vi "ImplementInterface.vi"(5 "AddInterfaceToClass(If not you still might want to create methods)":bool=TRUE, 6 "InterfaceMethodsToCreate":string[](array[string])=["Add.Vi", "Execute.vi"], 7 "ClassWriter.lvclass":refnum<class "ClassWriter.lvclass">, 8 "error in":errorcluster, 9 "CreateMethods":bool=TRUE, 10 "Interface Path":path=path "C:/Projects/Interface/Sub_Interface1/Sub_Interface1.lvclass", 11 "LvClassPath/LvClassProjectItem":variant) -> (0 "error out":errorcluster={"status"=TRUE, "code"=7, "source"="Invoke Node in InterfaceLibrary.lvlib:ImplementInterface.vi\n<APPEND>\nMethod Name: <b>LabVIEW Class:Open</b>"})   [LabVIEW 2020, in "InterfaceLibrary.lvlib"]
uses:
  InterfaceLibrary.lvlib
  Provider_BaseClassInterface/ClassWriter_class/ClassWriter.lvclass
  Provider_LvNativeClass/ClassWriterNative_class/ClassWriterNative.lvclass
  API/GDSAPI_SubVIs/GDSAPI_MethodType.ctl
  Provider_BaseClassInterface/CreateMethodData.ctl
  Provider_EndevoGOOP300/GOOP300_SubVIs/GOOP300_MethodScopeType.ctl
  Provider_LvNativeClass/ClassWriterNative_class/IconDetails.ctl
  Provider_LvNativeClass/ClassWriterNative_class/IconSize.ctl
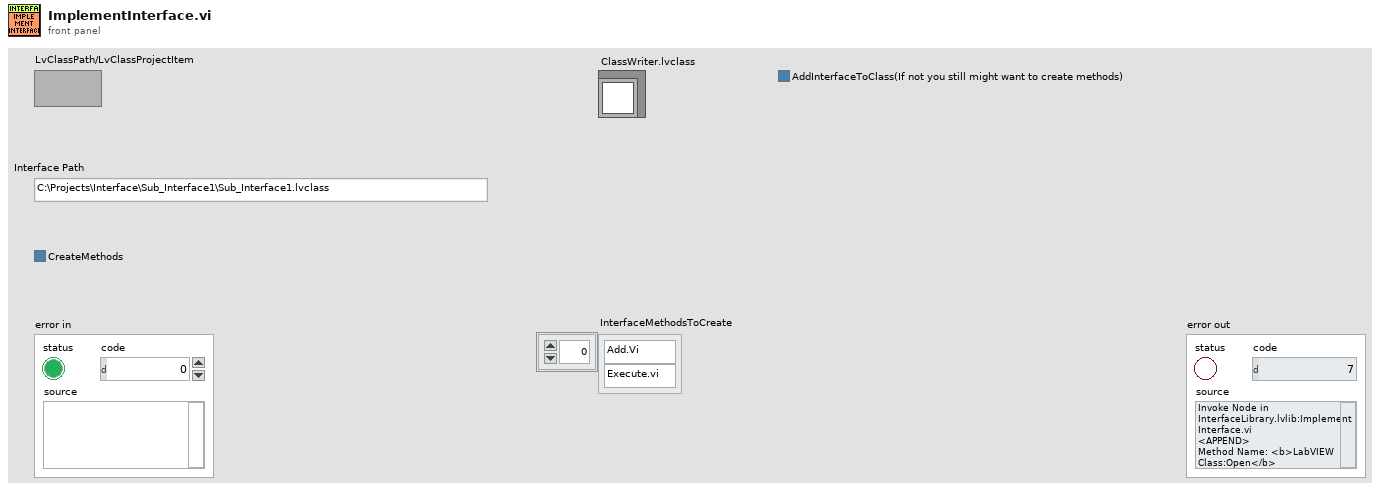
[diagram p1: front panel]
types:
  T1 = cluster{"ClassRef":refnum<vi>, "ClassRefCreated":bool, "Application":refnum<vi>, "InterfaceRef":refnum<vi>, "MethodsToImplement":path[], "MethodsDescription":string[], "MethodsScope":enum32{"invalid scope", "public", "private", "protected", "community"}[]}
  T2 = enum32{"invalid scope", "public", "private", "protected", "community"}
  T3 = typedef "GDSAPI_MethodType.ctl" = enum16{"Read Attribute", "Write Attribute", "Read & Write Attribute", "None Modifying Method", "Get Property", "Set Property", "Read Property", "Write Property", "Static Method", "Interface Method"}
  T4 = typedef "ClassWriter.lvclass/CreateMethodData.ctl" = cluster{"MethodName":string, "RelativeMethodPath":path, "MethodDescription":string, "Scope/Visibility":T5, "MethodTemplateName":string, "IconOut":u8[][], "RelativeProjectClassPath":string, "OpenViAfterCreation":bool, "DynamicDispatchVi":bool, "ExtraCreateParameters":variant, "MustOverride":bool, "MustCallParent":bool, "IconDetails":T6, "AF-Option":variant, "TemplatePath":path}
  T5 = typedef "GOOP300_MethodScopeType.ctl" = enum16{"Use Parent Folder Scope", "Public", "Protected", "Private", "Community"}
  T6 = typedef "ClassWriterNative.lvclass/IconDetails.ctl" = cluster{"IconSize":T7, "ImageRows(32)":i32, "ConnectorPaneHeight":i32[]}
  T7 = typedef "ClassWriterNative.lvclass/IconSize.ctl" = enum16{"Full", "1 c-term high", "2 c-term high", "3 c-term high"}
  T8 = enum32{"invalid scope", "public", "private", "protected", "community"}[]
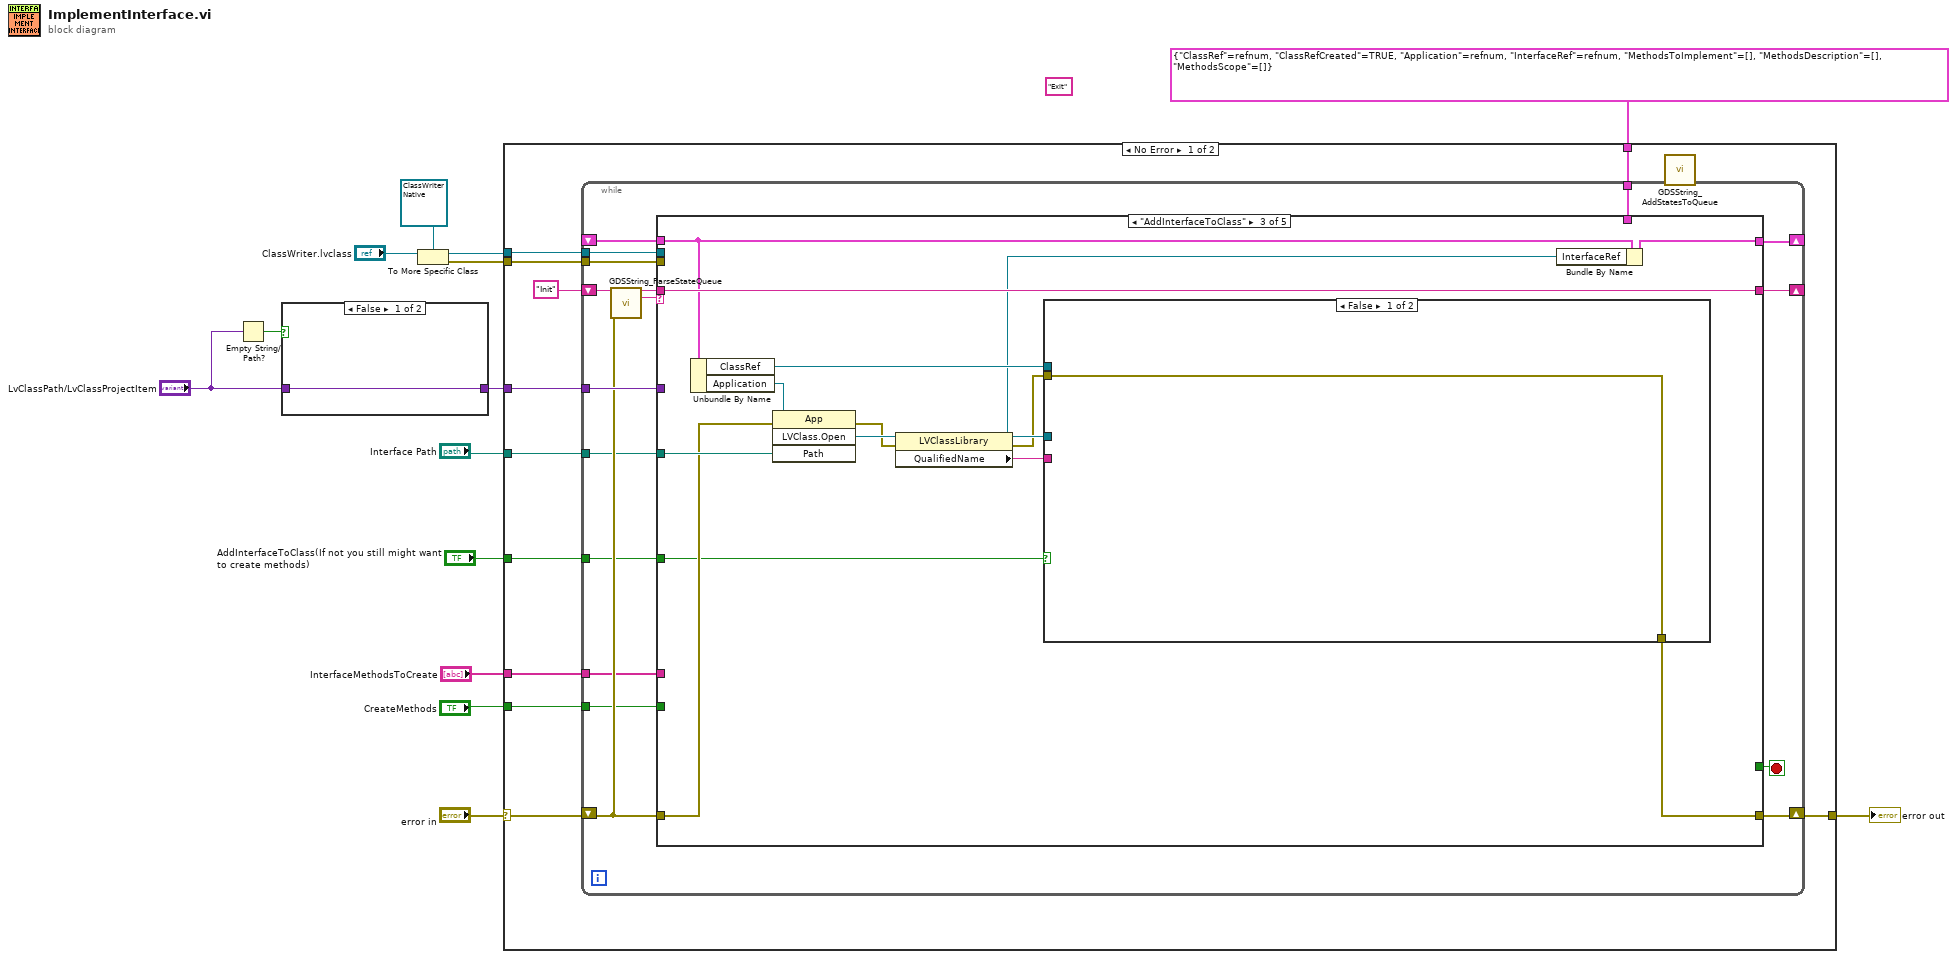
[diagram p0: block diagram]
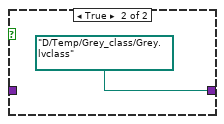
[diagram p2: hidden frame]
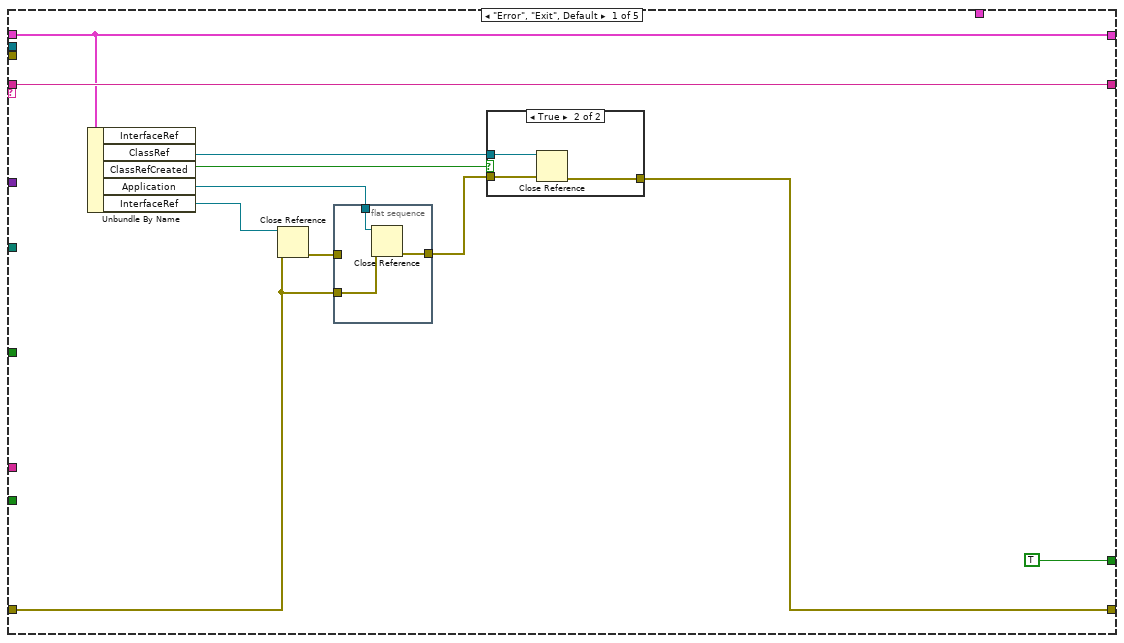
[diagram p3: hidden frame]
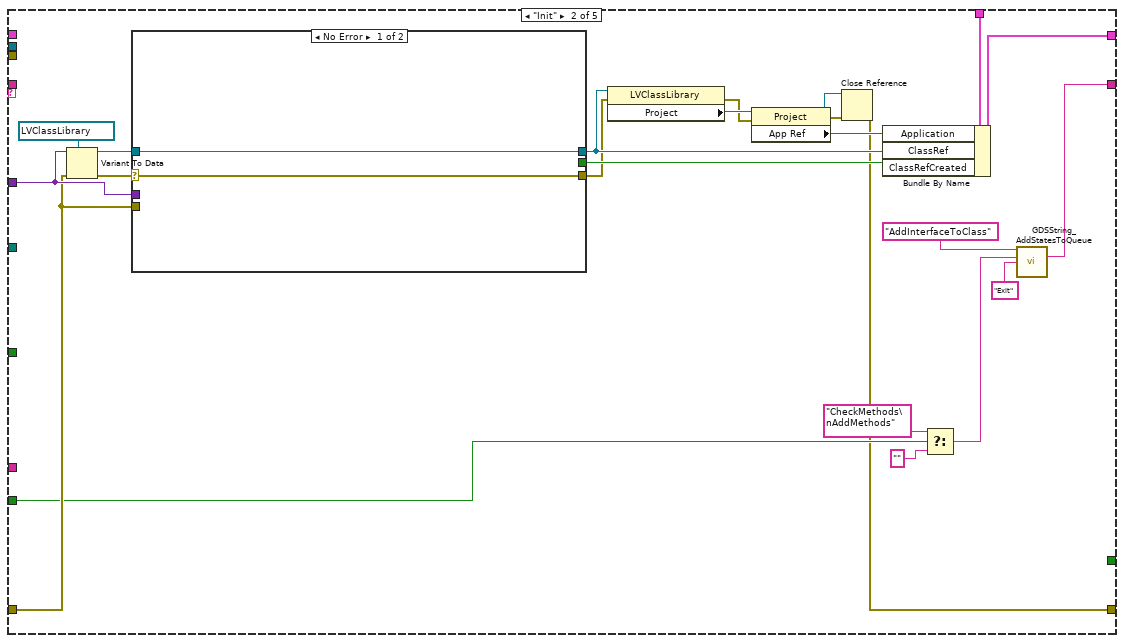
[diagram p5: hidden frame]
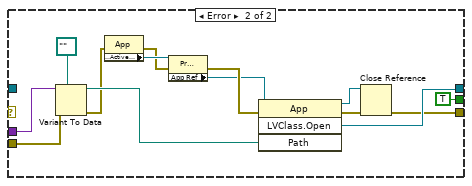
[diagram p6: hidden frame]
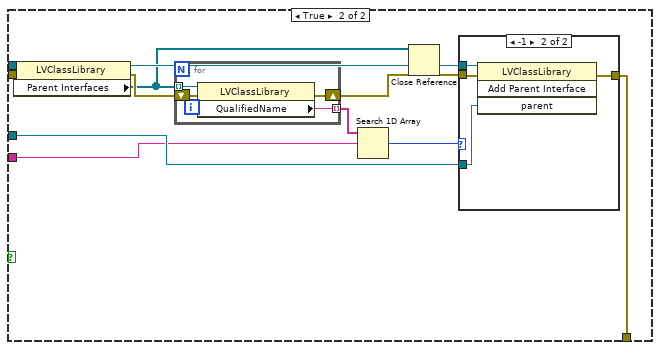
[diagram p7: hidden frame]
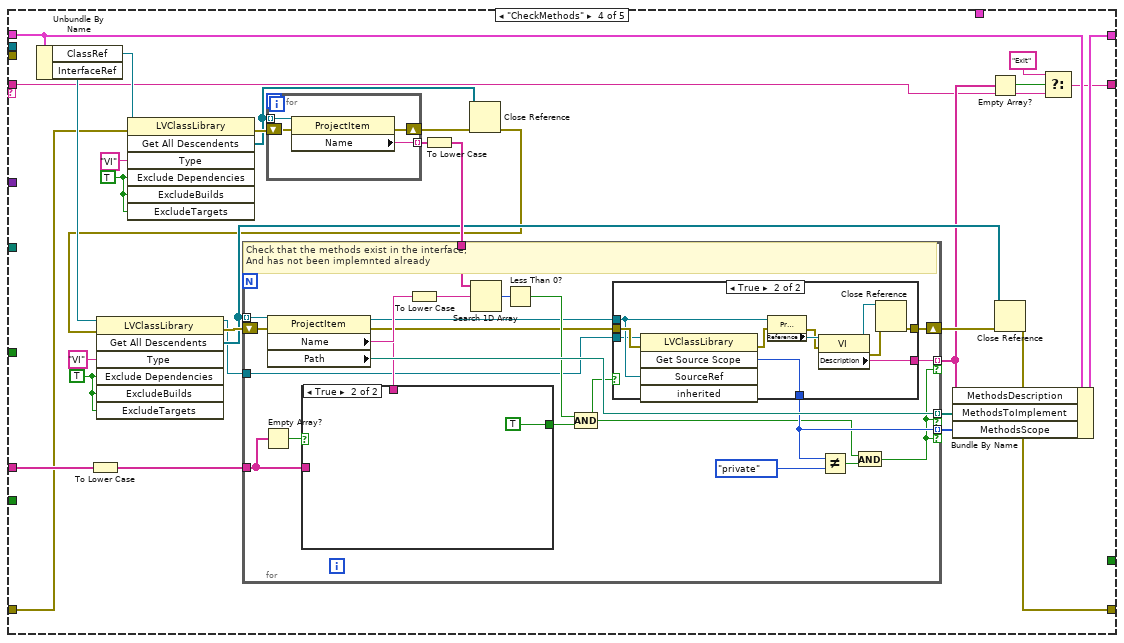
[diagram p9: hidden frame]
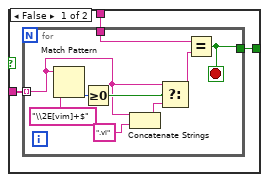
[diagram p11: hidden frame]
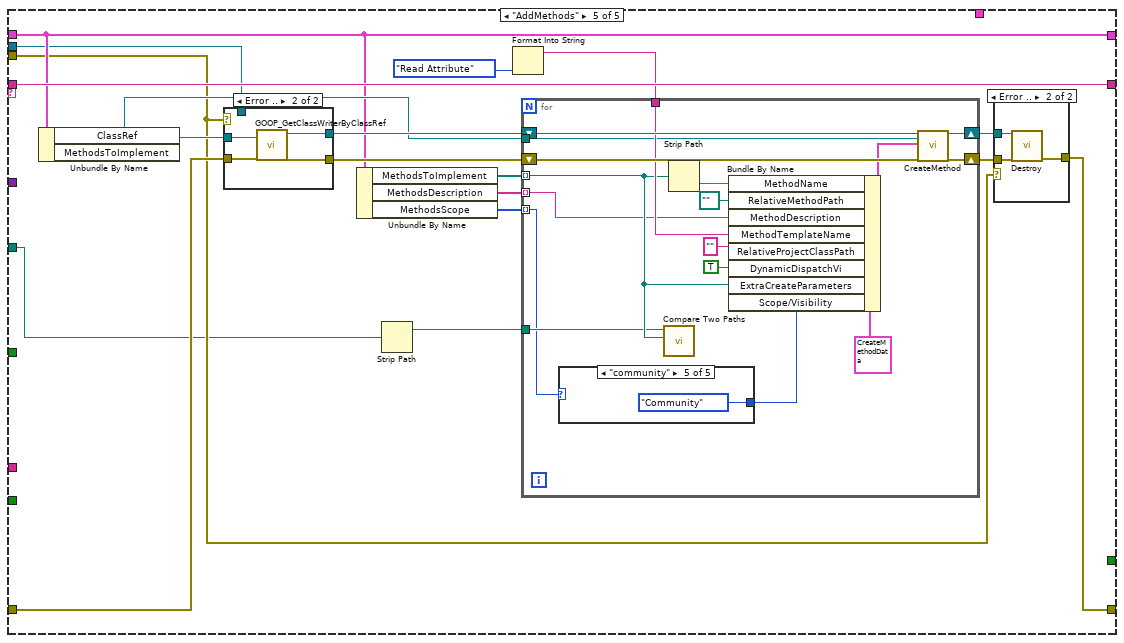
[diagram p12: hidden frame]
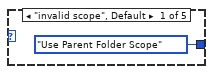
[diagram p15: hidden frame]
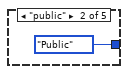
[diagram p16: hidden frame]
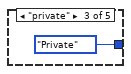
[diagram p17: hidden frame]
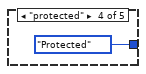
[diagram p18: hidden frame]
diagram:
  (unwired) "Exit" ("Remaining States")
  n1 = Empty String/Path?(string/path="LvClassPath/LvClassProjectItem") -> (empty?=w10:bool)
  n2 = case shown="False" w10 {
    tunnel: "LvClassPath/LvClassProjectItem" -> [w15 _]
    tunnel: [w15 path "D:/Temp/Grey_class/Grey.lvclass" ("Path")] -> w8
    frame False {
    }
    frame True {
    }
  }
  n3 = To More Specific Class(target class=refnum<class "ClassWriterNative.lvclass"> refnum ("ClassWriterNative"), reference="ClassWriter.lvclass") -> (specific class reference=w4:refnum<class "ClassWriterNative.lvclass">, error out=w2:errorcluster)  [unwired: 1 in]
  n4 = case shown="No Error" "error in" {
    selector: "error in" -> [w26 w267]
    tunnel: w8 -> [w27 _]
    tunnel: [w25 w267] -> w13
    tunnel: T1 {"ClassRef"=refnum, "ClassRefCreated"=TRUE, "Application"=refnum, "InterfaceRef"=refnum, "MethodsToImplement"=[], "MethodsDescription"=[], "MethodsScope"=[]} -> [w23 _]
    tunnel: "CreateMethods" -> [w22 _]
    tunnel: "Interface Path" -> [w21 _]
    tunnel: "InterfaceMethodsToCreate" -> [w20 _]
    tunnel: w4 -> [w19 _]
    tunnel: w2 -> [w18 _]
    tunnel: "AddInterfaceToClass(If not you still might want to create methods)" -> [w17 _]
    frame No Error {
      n5 = while {
        tunnel: w27 -> [w44]
        shift-right: [w43] -> w25
        shift-left: w26 -> [w41]
        shift-right: [w35] -> _
        shift-left: "Init" -> [w42]
        tunnel: w23 -> [w39]
        shift-right: [w38] -> _
        shift-left: _ -> [w37]
        tunnel: w22 -> [w33]
        tunnel: w21 -> [w32]
        tunnel: w20 -> [w31]
        tunnel: w19 -> [w30]
        tunnel: w18 -> [w29]
        tunnel: w17 -> [w28]
        stop <- w34 stop-if-true
        n6 = call "GDSString_ParseStateQueue.vi"("State Queue"=w42, "Error In (no error)"=w41) -> ("Remaining States"=w36:string, "Current State"=w40:string)  [unwired: 9 in, 3 out]
        n7 = case shown="\"AddInterfaceToClass\"" w40 {
          tunnel: w44 -> [_ w82 _ _ _]
          tunnel: w41 -> [w45 w81 w109 w145 w225]
          tunnel: [w48 w65 w110 w146 w229] -> w43
          tunnel: [w53 w79 w108 w155 w223] -> w38
          tunnel: w39 -> [_ w80 _ _ _]
          tunnel: w37 -> [w53 _ w114 w164 w223]
          tunnel: [w55 w77 w115 w153 w234] -> w35
          tunnel: w36 -> [w55 _ w115 w142 w234]
          tunnel: [TRUE _ _ _ _] -> w34
          tunnel: w33 -> [_ w76 _ _ _]
          tunnel: w32 -> [_ _ w111 _ w217]
          tunnel: w31 -> [_ _ _ w159 _]
          tunnel: w30 -> [_ _ _ _ w219]
          tunnel: w29 -> [_ _ _ _ w220]
          tunnel: w28 -> [_ _ w102 _ _]
          frame "Error", "Exit", Default {
            n8 = Unbundle By Name(w53) -> ("ClassRef"=w51:refnum<vi>, "ClassRefCreated"=w52:bool, "Application"=w50:refnum<vi>, "InterfaceRef"=w47:refnum<vi>)  [unwired: 1 out]
            n9 = Close Reference(reference=w47, error in (no error)=w45) -> (error out=w46:errorcluster)
            n10 = flat-sequence {
              tunnel: w50 -> [w58]
              tunnel: [w57] -> w49
              tunnel: w46 -> [_]
              tunnel: w45 -> [w56]
              frame #0 {
                n11 = Close Reference(reference=w58, error in (no error)=w56) -> (error out=w57:errorcluster)
              }
            }
            n12 = case shown="True" w52 {
              tunnel: w51 -> [_ w62]
              tunnel: w49 -> [w59 w61]
              tunnel: [w59 w60] -> w48
              frame False {
              }
              frame True {
                n13 = Close Reference(reference=w62, error in (no error)=w61) -> (error out=w60:errorcluster)
              }
            }
          }
          frame "Init" {
            n14 = Variant To Data(error in=w81, type=refnum<vi> refnum ("ProjectItem"), Variant=w82) -> (data=w84:refnum<vi>, error out=w83:errorcluster)
            n15 = case shown="No Error" w83 {
              selector: w83 -> [w86 _]
              tunnel: w84 -> [w87 _]
              tunnel: [w86 w93] -> w66
              tunnel: w82 -> [_ w100]
              tunnel: w81 -> [_ w97]
              tunnel: [w87 w96] -> w70
              tunnel: [_ TRUE] -> w78
              frame No Error {
              }
              frame Error {
                n16 = Variant To Data(error in=w97, type=path "" ("Path"), Variant=w100) -> (data=w99:path, error out=w98:errorcluster)
                n17 = property class="App"(error in=w98) -> (error out=w90:errorcluster, "Project.ActiveProject"=w91:refnum<vi>)  [unwired: 1 in, 1 out]
                n18 = property class="Project"(reference=w91, error in=w90) -> (error out=w89:errorcluster, "App Ref"=w88:refnum<vi>)  [unwired: 1 out]
                n19 = invoke class="App" method="LVClass.Open"(reference=w88, error in=w89, "Path"=w99) -> (reference out=w94:refnum<vi>, error out=w95:errorcluster, "LVClass.Open"=w96:refnum<vi>)  [unwired: 1 in, 1 out]
                n20 = Close Reference(reference=w94, error in (no error)=w95) -> (error out=w93:errorcluster)
              }
            }
            n21 = property class="LVClassLibrary"(reference=w70, error in=w66) -> (error out=w63:errorcluster, "Project"=w64:refnum<vi>)  [unwired: 1 out]
            n22 = property class="Project"(reference=w64, error in=w63) -> (reference out=w68:refnum<vi>, error out=w67:errorcluster, "App Ref"=w69:refnum<vi>)
            n23 = Close Reference(reference=w68, error in (no error)=w67) -> (error out=w65:errorcluster)
            n24 = Bundle By Name(cluster=w80, "Application"=w69, "ClassRef"=w70, "ClassRefCreated"=w78) -> (w79:T1)
            n25 = Select(t="CheckMethods\nAddMethods" ("Remaining States"), s=w76, f="") -> (s? t:f=w72:string)
            n26 = call "GDSString_AddStatesToQueue.vi"("State(s) in Front (\"\")"="AddInterfaceToClass" ("Remaining States"), "State(s) in (\"\")"=w72, "State(s) at Back (\"\")"="Exit" ("Remaining States")) -> ("States Out"=w77:string)  [unwired: 12 in]
          }
          frame "AddInterfaceToClass" {
            n27 = Unbundle By Name(w114) -> ("ClassRef"=w113:refnum<vi>, "Application"=w112:refnum<vi>)
            n28 = invoke class="App" method="LVClass.Open"(reference=w112, error in=w109, "Path"=w111) -> (error out=w104:errorcluster, "LVClass.Open"=w107:refnum<vi>)  [unwired: 1 in, 2 out]
            n29 = property class="LVClassLibrary"(reference=w107, error in=w104) -> (reference out=w106:refnum<vi>, error out=w103:errorcluster, "QualifiedName"=w105:string)
            n30 = case shown="False" w102 {
              tunnel: w113 -> [_ w128]
              tunnel: [w116 w125] -> w110
              tunnel: w106 -> [_ w124]
              tunnel: w105 -> [_ w123]
              tunnel: w103 -> [w116 w122]
              frame False {
              }
              frame True {
                n31 = property class="LVClassLibrary"(reference=w128, error in=w122) -> (reference out=w126:refnum<vi>, error out=w121:errorcluster, "Parent Interfaces"=w117:refnum<vi>[])
                n32 = for {
                  tunnel: w117 -> [w132] mode=indexing
                  tunnel: [w131] -> w120 mode=indexing
                  shift-right: [w130] -> w119
                  shift-left: w121 -> [w129]
                  n33 = property class="LVClassLibrary"(reference=w132, error in=w129) -> (error out=w130:errorcluster, "QualifiedName"=w131:string)  [unwired: 1 out]
                }
                n34 = Search 1D Array(1D array=w120, element=w123) -> (index of element=w127:i32)  [unwired: 1 in]
                n35 = Close Reference(reference=w117, error in (no error)=w119) -> (error out=w118:errorcluster)
                n36 = case shown="-1" w127 {
                  tunnel: w126 -> [_ w137]
                  tunnel: w118 -> [w133 w136]
                  tunnel: w124 -> [_ w135]
                  tunnel: [w133 w134] -> w125
                  frame 0, Default {
                  }
                  frame -1 {
                    n37 = invoke class="LVClassLibrary" method="Add Parent Interface"(reference=w137, error in=w136, "parent"=w135) -> (error out=w134:errorcluster)  [unwired: 1 in, 3 out]
                  }
                }
              }
            }
            n38 = Bundle By Name(cluster=w114, "InterfaceRef"=w106) -> (w108:T1)
          }
          frame "CheckMethods" {
            w162 = TRUE ("ExcludeDependencies")
            w165 = TRUE ("ExcludeDependencies")
            n39 = Unbundle By Name(w164) -> ("ClassRef"=w163:refnum<vi>, "InterfaceRef"=w160:refnum<vi>)
            n40 = To Lower Case(string=w159) -> (all lower case string=w158:string[])
            n41 = invoke class="LVClassLibrary" method="Get All Descendents"(reference=w163, error in=w145, "Type"="VI", "Exclude Dependencies"=w165, "ExcludeBuilds"=w165, "ExcludeTargets"=w165) -> (error out=w166:errorcluster, "All Descendents"=w147:refnum<vi>[])  [unwired: 1 in, 5 out]
            n42 = for {
              tunnel: w147 -> [w216] mode=indexing
              tunnel: [w215] -> w157 mode=indexing
              shift-right: [w213] -> w149
              shift-left: w166 -> [w214]
              n43 = property class="ProjectItem"(reference=w216, error in=w214) -> (error out=w213:errorcluster, "Name"=w215:string)  [unwired: 1 out]
            }
            n44 = To Lower Case(string=w157) -> (all lower case string=w156:string[])
            n45 = Close Reference(reference=w147, error in (no error)=w149) -> (error out=w148:errorcluster)
            n46 = invoke class="LVClassLibrary" method="Get All Descendents"(reference=w160, error in=w148, "Type"="VI", "Exclude Dependencies"=w162, "ExcludeBuilds"=w162, "ExcludeTargets"=w162) -> (reference out=w140:refnum<vi>, error out=w161:errorcluster, "All Descendents"=w150:refnum<vi>[])  [unwired: 1 in, 4 out]
            n47 = for {
              tunnel: w150 -> [w187] mode=indexing
              shift-right: [w174] -> w151
              shift-left: w161 -> [w186]
              tunnel: [w185] -> w144 mode=indexing if=w167
              tunnel: w158 -> [w183]
              tunnel: w156 -> [w179]
              tunnel: [w173] -> w143 mode=indexing if=w167
              tunnel: [w171] -> w141 mode=indexing if=w167
              tunnel: w140 -> [w172]
              # "Check that the methods exist in the interface,\nAnd has not been implemnted already"
              n48 = Empty Array?(array=w183) -> (empty?=w181:bool)
              n49 = property class="ProjectItem"(reference=w187, error in=w186) -> (reference out=w175:refnum<vi>, error out=w176:errorcluster, "Name"=w184:string, "Path"=w185:path)
              n50 = To Lower Case(string=w184) -> (all lower case string=w180:string)
              n51 = case shown="True" w181 {
                tunnel: w180 -> [w202 _]
                tunnel: w183 -> [w201 _]
                tunnel: [w200 TRUE] -> w182
                frame False {
                  n52 = for {
                    tunnel: [w203] -> w200
                    tunnel: w202 -> [w206]
                    tunnel: w201 -> [w205] mode=indexing
                    stop <- w203 stop-if-true
                    n53 = Match Pattern(string=w205, regular expression="\\2E[vim]+$") -> (offset past match=w210:i32)  [unwired: 1 in, 3 out]
                    n54 = Greater Or Equal To 0?(x=w210) -> (x >= 0?=w209:bool)
                    n55 = Concatenate Strings(w205, ".vi" ("string")) -> (w208:string)
                    n56 = Select(t=w205, s=w209, f=w208) -> (s? t:f=w204:string)
                    n57 = Equal?(x=w206, y=w204) -> (x = y?=w203:bool)
                  }
                }
                frame True {
                }
              }
              n58 = Search 1D Array(1D array=w179, element=w180) -> (index of element=w178:i32)  [unwired: 1 in]
              n59 = Less Than 0?(x=w178) -> (x < 0?=w177:bool)
              n60 = Compound Arithmetic op=AND(w177, w182) -> (w168:bool)
              n61 = case shown="True" w168 {
                tunnel: w176 -> [w188 w192]
                tunnel: w175 -> [_ w191]
                tunnel: [w188 w194] -> w174
                tunnel: [_ w197] -> w173
                tunnel: [_ w190] -> w171
                tunnel: w172 -> [_ w189]
                frame False {
                }
                frame True {
                  n62 = invoke class="LVClassLibrary" method="Get Source Scope"(reference=w189, error in=w192, "SourceRef"=w191) -> (error out=w193:errorcluster, "GetSourceScope"=w190:T2)  [unwired: 2 in, 3 out]
                  n63 = property class="ProjectItem"(reference=w191, error in=w193) -> (error out=w198:errorcluster, "Reference"=w199:refnum<vi>)  [unwired: 1 out]
                  n64 = property class="VI"(reference=w199, error in=w198) -> (reference out=w196:refnum<vi>, error out=w195:errorcluster, "Description"=w197:string)
                  n65 = Close Reference(reference=w196, error in (no error)=w195) -> (error out=w194:errorcluster)
                }
              }
              n66 = Not Equal?(x=w171, y=T2."private") -> (x != y?=w169:bool)
              n67 = And(x=w168, y=w169) -> (x .and. y?=w167:bool)
            }
            n68 = Bundle By Name(cluster=w164, "MethodsDescription"=w143, "MethodsToImplement"=w144, "MethodsScope"=w141) -> (w155:T1)
            n69 = Empty Array?(array=w143) -> (empty?=w154:bool)
            n70 = Close Reference(reference=w150, error in (no error)=w151) -> (error out=w146:errorcluster)
            n71 = Select(t="Exit" ("Remaining States"), s=w154, f=w142) -> (s? t:f=w153:string)
          }
          frame "AddMethods" {
            n72 = Unbundle By Name(w223) -> ("ClassRef"=w226:refnum<vi>)  [unwired: 1 out]
            n73 = case shown="Error .." w220 {
              tunnel: w226 -> [_ w244]
              tunnel: [w240 w243] -> w233
              tunnel: [w239 w242] -> w232
              tunnel: w219 -> [w240 _]
              tunnel: w225 -> [w239 w241]
              frame No Error {
              }
              frame Error {
                n74 = call "GOOP_GetClassWriterByClassRef.vi"("LVClassLibrary Refnum"=w244, "error in (no error)"=w241) -> ("ClassWriterNative.lvclass"=w243:refnum<class "ClassWriterNative.lvclass">, "error out"=w242:errorcluster)  [unwired: 16 in]
              }
            }
            n75 = Unbundle By Name(w223) -> ("MethodsToImplement"=w224:path[], "MethodsDescription"=w222:string[], "MethodsScope"=w221:T8)
            n76 = Strip Path(path=w217) -> (stripped path=w218:path)  [unwired: 1 out]
            n77 = Format Into String(GDSAPI_MethodType."Read Attribute" ("MethodType")) -> (resulting string=w227:string)  [unwired: 3 in, 1 out]
            n78 = for {
              shift-right: [w259] -> w231
              shift-left: w233 -> [w261]
              shift-right: [w258] -> w230
              shift-left: w232 -> [w260]
              tunnel: w227 -> [w257]
              tunnel: w224 -> [w256] mode=indexing
              tunnel: w218 -> [w255]
              tunnel: w226 -> [w254]
              tunnel: w222 -> [w248] mode=indexing
              tunnel: w221 -> [w247] mode=indexing
              n79 = case shown="\"community\"" w247 {
                tunnel: [GOOP300_MethodScopeType."Use Parent Folder Scope" ("Scope/Visibility") GOOP300_MethodScopeType."Public" ("Scope/Visibility") GOOP300_MethodScopeType."Private" ("Scope/Visibility") GOOP300_MethodScopeType."Protected" ("Scope/Visibility") GOOP300_MethodScopeType."Community" ("Scope/Visibility")] -> w246
                frame "invalid scope", Default {
                }
                frame "public" {
                }
                frame "private" {
                }
                frame "protected" {
                }
                frame "community" {
                }
              }
              n80 = call <vilib>:"Compare Two Paths.vi"("Path 2"=w256, "Path 1"=w255) -> ()  [unwired: 6 in, 4 out]
              n81 = Strip Path(path=w256) -> (name=w250:string)  [unwired: 1 out]
              n82 = Bundle By Name(cluster=T4 {"MethodName"="", "RelativeMethodPath"=path "", "MethodDescription"="", "Scope/Visibility"=enum."Use Parent Folder Scope", "MethodTemplateName"="", "IconOut"=[], "RelativeProjectClassPath"="", "OpenViAfterCreation"=FALSE, "DynamicDispatchVi"=FALSE, "ExtraCreateParameters"=variant, "MustOverride"=FALSE, "MustCallParent"=FALSE, "IconDetails"={"IconSize"=enum."Full", "ImageRows(32)"=0, "ConnectorPaneHeight"=[]}, "AF-Option"=variant, "TemplatePath"=path ""} ("CreateMethodData"), "MethodName"=w250, "RelativeMethodPath"=path "", "MethodDescription"=w248, "MethodTemplateName"=w257, "RelativeProjectClassPath"="", "DynamicDispatchVi"=TRUE, "ExtraCreateParameters"=w256, "Scope/Visibility"=w246) -> (w251:T4)
              n83 = call-dynamic "CreateMethod.vi"("ClassWriterNative.lvclass"=w261, "ClassItemRefIn"=w254, "CreateMethodData"=w251, "error in (no error)"=w260) -> ("ClassWriterNative.lvclass 2"=w259:refnum<class "ClassWriterNative.lvclass">, "error out"=w258:errorcluster)  [unwired: 12 in, 2 out]
            }
            n84 = case shown="Error .." w220 {
              tunnel: w231 -> [_ w238]
              tunnel: w230 -> [w235 w237]
              tunnel: [w235 w236] -> w229
              frame No Error {
              }
              frame Error {
                n85 = call-dynamic "Destroy.vi"("ClassWriterNative"=w238, "error in (no error)"=w237) -> ("error out"=w236:errorcluster)  [unwired: 17 in]
              }
            }
          }
        }
      }
      n86 = call "GDSString_AddStatesToQueue.vi"() -> ()  [unwired: 15 in, 1 out]
    }
    frame Error {
    }
  }
  "error out" <- w13
